vi "Get Minimum Trigger Interval.vi"(8 "error in (no error)":errorcluster, 11 "Abstract DAQ Triggered Actor in":refnum<class "Abstract DAQ Triggered Actor.lvclass">) -> (0 "error out":errorcluster, 2 "Minimum Interval (ms)":dbl, 3 "Abstract DAQ Triggered Actor out":refnum<class "Abstract DAQ Triggered Actor.lvclass">)   [LabVIEW 2020, in "DAQ Timed SPIM.lvlib" / "Abstract DAQ Triggered Actor.lvlib" / "Abstract DAQ Triggered Actor.lvclass"]
uses:
  Abstract DAQ Triggered Actor.lvclass
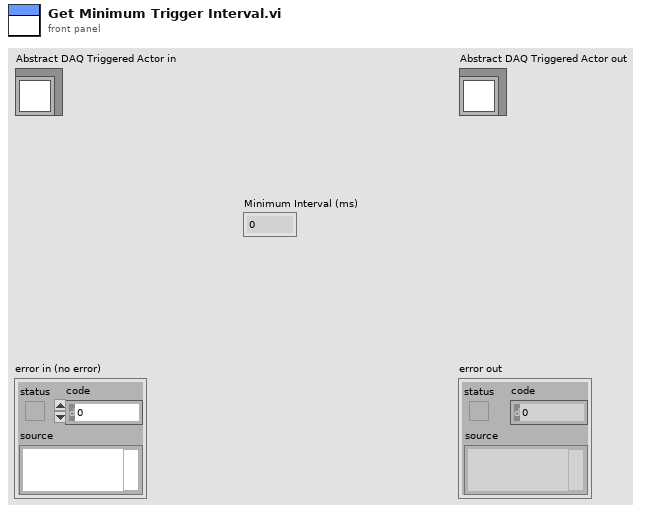
[diagram p1: front panel]
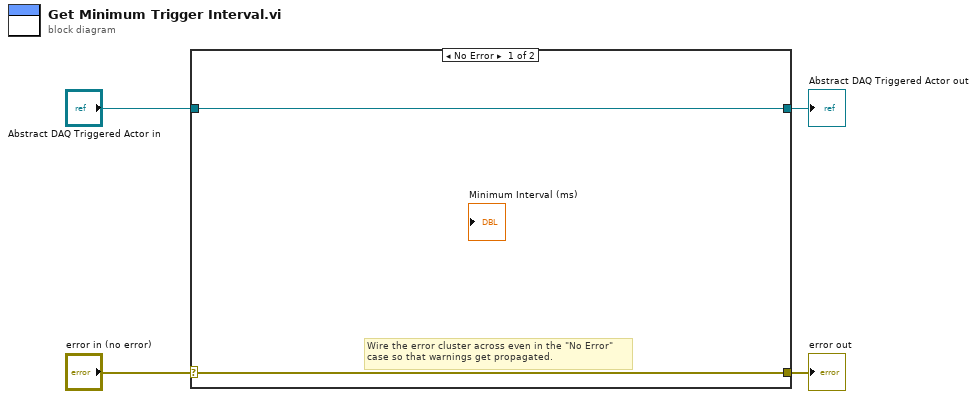
[diagram p0: block diagram]
diagram:
  n1 = case shown="No Error" "error in (no error)" {
    selector: "error in (no error)" -> [w5 w8]
    tunnel: [w5 w8] -> w3
    tunnel: [w6 w7] -> w1
    tunnel: "Abstract DAQ Triggered Actor in" -> [w6 w7]
    frame No Error {
      # "Wire the error cluster across even in the \"No Error\"\ncase so that warnings get propagated."
    }
    frame Error {
    }
  }
  "error out" <- w3
  "Abstract DAQ Triggered Actor out" <- w1
